vi "SC Copy Robot Project.vi"(8 "error in (no error)":errorcluster, 9 "target":string, 10 "root":string, 11 "name":string) -> (0 "error out":errorcluster, 1 "opened?":bool)   [LabVIEW 2023]
doc: "Copies one of a robot's projects (root, its root commit; name) to this computer and opens it, as Open Deployed Project does: in the robot's own IDE into ~/Projects/<name> (reusing an existing copy), on a desktop into a new folder the user creates. Shows the result first; opened? is true when a project was opened."
uses:
  <vilib>/Utility/sysdir.llb/System Directory Type.ctl
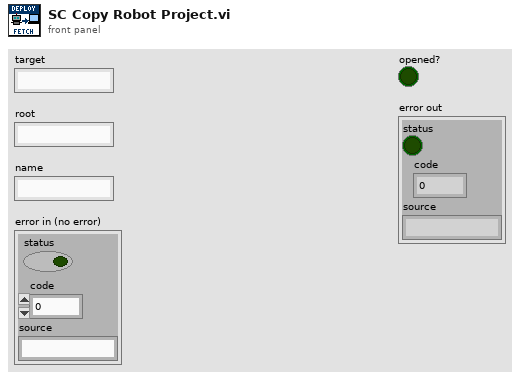
[diagram p1: front panel]
types:
  T1 = typedef "System Directory Type.ctl" = i32
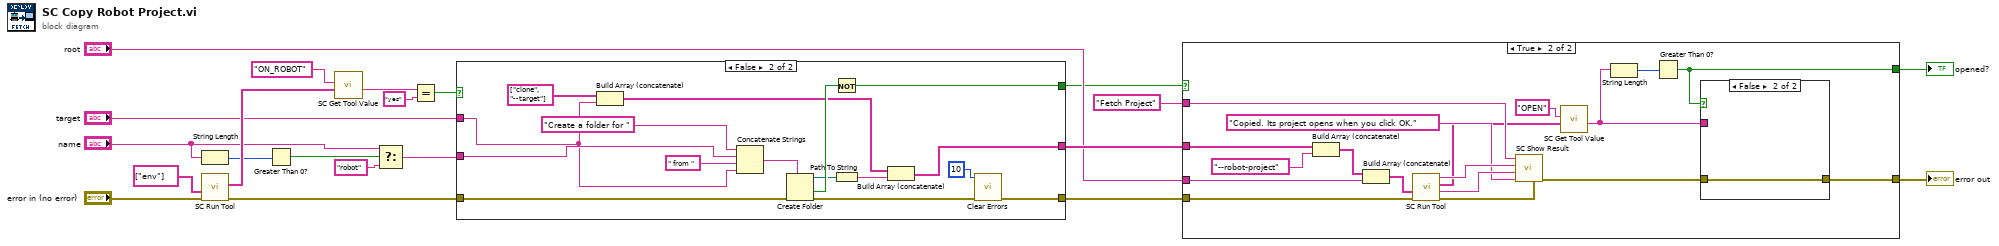
[diagram p0: block diagram]
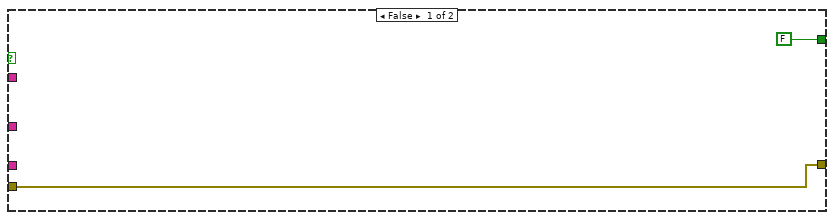
[diagram p2: hidden frame]
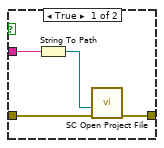
[diagram p3: hidden frame]
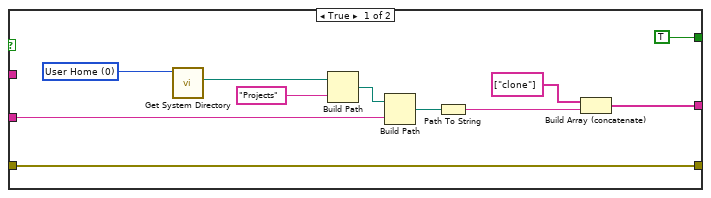
[diagram p4: hidden frame]
diagram:
  n1 = String Length(string="name") -> (length=w15:i32)
  n2 = call "SC Run Tool.vi"("error in (no error)"="error in (no error)", "arguments"=string[] ["env"]) -> ("error out"=w11:errorcluster, "tool lines"=w19:string[])  [unwired: 4 in, 4 out]
  n3 = Greater Than 0?(x=w15) -> (x > 0?=w14:bool)
  n4 = call "SC Get Tool Value.vi"("tool lines"=w19, "key"="ON_ROBOT") -> ("value"=w17:string)  [unwired: 8 in, 1 out]
  n5 = Select(t="name", s=w14, f="robot") -> (s? t:f=w10:string)
  n6 = Equal?(x=w17, y="yes") -> (x = y?=w8:bool)
  n7 = case shown="False" w8 {
    tunnel: w11 -> [w22 w45]
    tunnel: w10 -> [w28 w47]
    tunnel: "target" -> [_ w38]
    tunnel: [TRUE w35] -> w1
    tunnel: [w23 w34] -> w7
    tunnel: [w22 w33] -> w6
    frame True {
      w32 = T1 0 items=["User Home"=0, "User Desktop"=1, "User Documents"=2, "User Application Data"=3, "User Preferences"=4, "User Temporary"=5, "Public Documents"=6, "Public Application Data"=7, "Public Preferences"=8, "Public Cache"=13, "System Core Libraries"=9, "System Installed Libraries"=10, "Application Files"=11, "Boot Volume Root"=12]
      n8 = call <vilib>:"Get System Directory.vi"("system directory type"=w32) -> ("system directory"=w31:path)  [unwired: 10 in]
      n9 = Build Path(base path=w31, name or relative path="Projects") -> (appended path=w29:path)
      n10 = Build Path(base path=w29, name or relative path=w28) -> (appended path=w27:path)
      n11 = Path To String(path=w27) -> (string=w25:string)
      n12 = Build Array (concatenate)(string[] ["clone"], w25) -> (w23:string[])
    }
    frame False {
      n13 = Build Array (concatenate)(string[] ["clone", "--target"], w38) -> (w37:string[])
      n14 = Concatenate Strings("Create a folder for ", w47, " from ", w38) -> (w44:string)
      n15 = Create Folder(prompt (Create Folder)=w44, error in=w45) -> (created path=w40:path, cancelled=w41:bool, error out=w43:errorcluster)  [unwired: 1 in]
      n16 = Not(x=w41) -> (.not. x?=w35:bool)
      n17 = Path To String(path=w40) -> (string=w36:string)
      n18 = Build Array (concatenate)(w37, w36) -> (w34:string[])
      n19 = call <vilib>:"Clear Errors.vi"("error in (no error)"=w43, "specific error code to clear (0: all)"=10) -> ("error out"=w33:errorcluster)  [unwired: 4 in, 1 out]
    }
  }
  n20 = case shown="True" w1 {
    tunnel: w7 -> [_ w68]
    tunnel: w6 -> [w50 w63]
    tunnel: "root" -> [_ w65]
    tunnel: "Fetch Project" -> [_ w60]
    tunnel: [w50 w52] -> w3
    tunnel: [FALSE w51] -> w2
    frame False {
    }
    frame True {
      n21 = Build Array (concatenate)(w68, "--robot-project") -> (w66:string[])
      n22 = Build Array (concatenate)(w66, w65) -> (w64:string[])
      n23 = call "SC Run Tool.vi"("error in (no error)"=w63, "arguments"=w64) -> ("error out"=w58:errorcluster, "output"=w62:string, "tool lines"=w57:string[], "result"=w61:string)  [unwired: 4 in, 2 out]
      n24 = call "SC Show Result.vi"("error in (no error)"=w58, "OK message"="Copied. Its project opens when you click OK.", "output"=w62, "result"=w61, "title"=w60) -> ("error out"=w53:errorcluster)  [unwired: 6 in]
      n25 = call "SC Get Tool Value.vi"("tool lines"=w57, "key"="OPEN") -> ("value"=w54:string)  [unwired: 8 in, 1 out]
      n26 = String Length(string=w54) -> (length=w55:i32)
      n27 = Greater Than 0?(x=w55) -> (x > 0?=w51:bool)
      n28 = case shown="False" w51 {
        tunnel: w54 -> [w72 _]
        tunnel: w53 -> [w70 w73]
        tunnel: [w69 w73] -> w52
        frame True {
          n29 = String To Path(string=w72) -> (path=w71:path)
          n30 = call "SC Open Project File.vi"("error in (no error)"=w70, "path"=w71) -> ("error out"=w69:errorcluster)  [unwired: 9 in]
        }
        frame False {
        }
      }
    }
  }
  "opened?" <- w2
  "error out" <- w3
